vi "Get Multi-Line Package Attribute Value.vi"(8 "error in (no error)":errorcluster, 10 "package attribute name":string, 11 "package attributes CLI string":string) -> (0 "error out":errorcluster, 1 "attribute found?":bool, 2 "description":string, 3 "synopsis":string)   [LabVIEW 2014, in "NIPM_API.lvlib"]
doc: "Gets the synopsis and description values for a multi-line attribute in a package attribute string.\n\nINPUT(s)\n<B>Package attributes string in</B>: This is the initial string containing the package attributes and values. For example, this string could come from the output of a nipkg CLI command.\n\n<B>Package attribute name</B>: This is the name of the attribute whose value you want to change.\n\nOUTPUT(s)\n<B>Synopsis</B>: Returns the synopsis value of the multi-line package attribute\n\n<B>Description</B>: Returns the description value of the multi-line package attribute\n\n<B>Attribute found?</B>: Returns whether the attribute was found"
uses:
  NIPM_API.lvlib
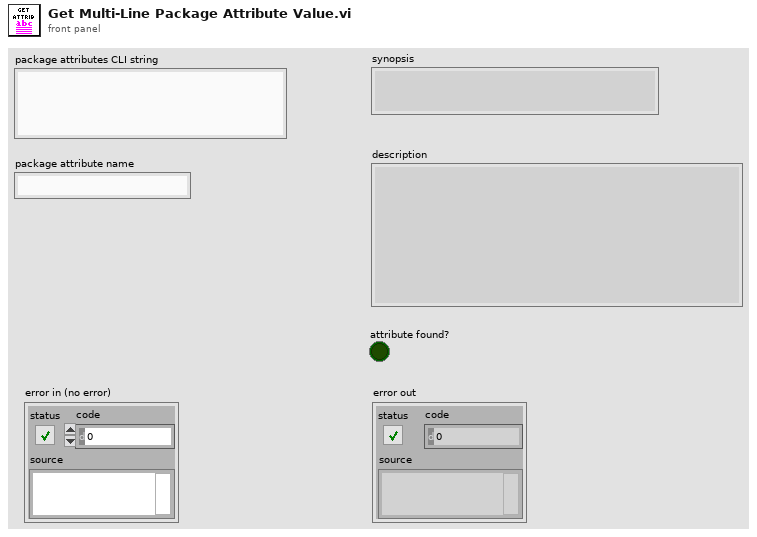
[diagram p1: front panel]
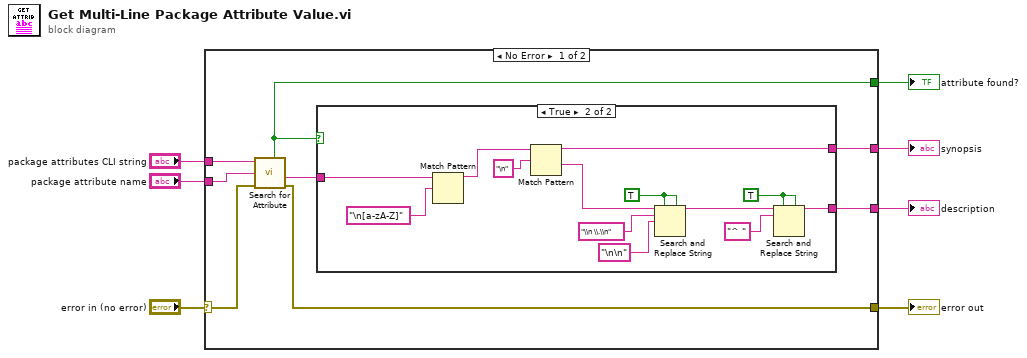
[diagram p0: block diagram]
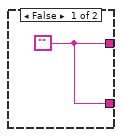
[diagram p2: hidden frame]
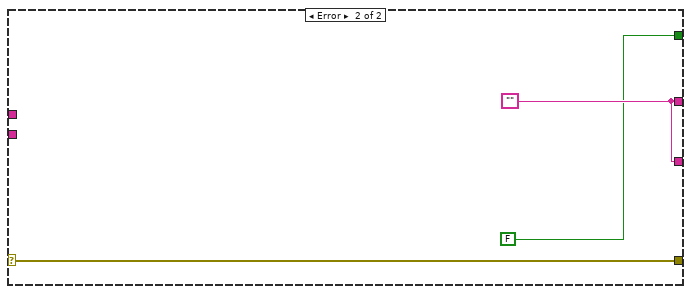
[diagram p3: hidden frame]
diagram:
  n1 = case shown="No Error" "error in (no error)" {
    selector: "error in (no error)" -> [w11 w32]
    tunnel: "package attributes CLI string" -> [w13 _]
    tunnel: "package attribute name" -> [w12 _]
    tunnel: [w15 w31] -> w6
    tunnel: [w10 w32] -> w4
    tunnel: [w14 w31] -> w3
    tunnel: [w9 FALSE] -> w1
    frame No Error {
      n2 = call "Search for Attribute.vi"("error in (no error)"=w11, "package attribute name"=w12, "package attributes CLI string in"=w13) -> ("error out"=w10:errorcluster, "string after attribute"=w8:string, "attribute found?"=w9:bool)  [unwired: 3 in, 3 out]
      n3 = case shown="True" w9 {
        tunnel: w8 -> [_ w29]
        tunnel: [w16 w25] -> w15
        tunnel: [w16 w20] -> w14
        frame False {
          w16 = ""
        }
        frame True {
          w22 = TRUE ("replace all? (F)")
          w24 = TRUE ("replace all? (F)")
          n4 = Match Pattern(string=w29, regular expression="\n[a-zA-Z]" ("Package Attribute Name")) -> (before substring=w26:string)  [unwired: 1 in, 3 out]
          n5 = Match Pattern(string=w26, regular expression="\n") -> (before substring=w25:string, after substring=w23:string)  [unwired: 1 in, 2 out]
          n6 = Search and Replace String(replace all?=w24, multiline?=w24, input string=w23, search string="\\n \\.\\n", replace string="\n\n" ("search string")) -> (result string=w19:string)  [unwired: 3 in, 3 out]
          n7 = Search and Replace String(replace all?=w22, multiline?=w22, input string=w19, search string="^ ") -> (result string=w20:string)  [unwired: 4 in, 3 out]
        }
      }
    }
    frame Error {
      w31 = ""
    }
  }
  "synopsis" <- w6
  "error out" <- w4
  "description" <- w3
  "attribute found?" <- w1
